vi "elevator_TP.vi"() -> ()   [LabVIEW 2020]
uses:
  State_enum.ctl
panel:
  out "Going down":bool
  out "Going up":bool
  out "Door closed":bool
  out "Alarm":bool
  out "Door open":bool
  out "Motor":bool
  out "state":T1
  in  "Stop Button":bool
  in  "1":bool
  in  "2":bool
  in  "3":bool
  out "Elevator":i8(slide) scale=0.0..2.0
  out "Destination floor":i32
  # "Current floor"
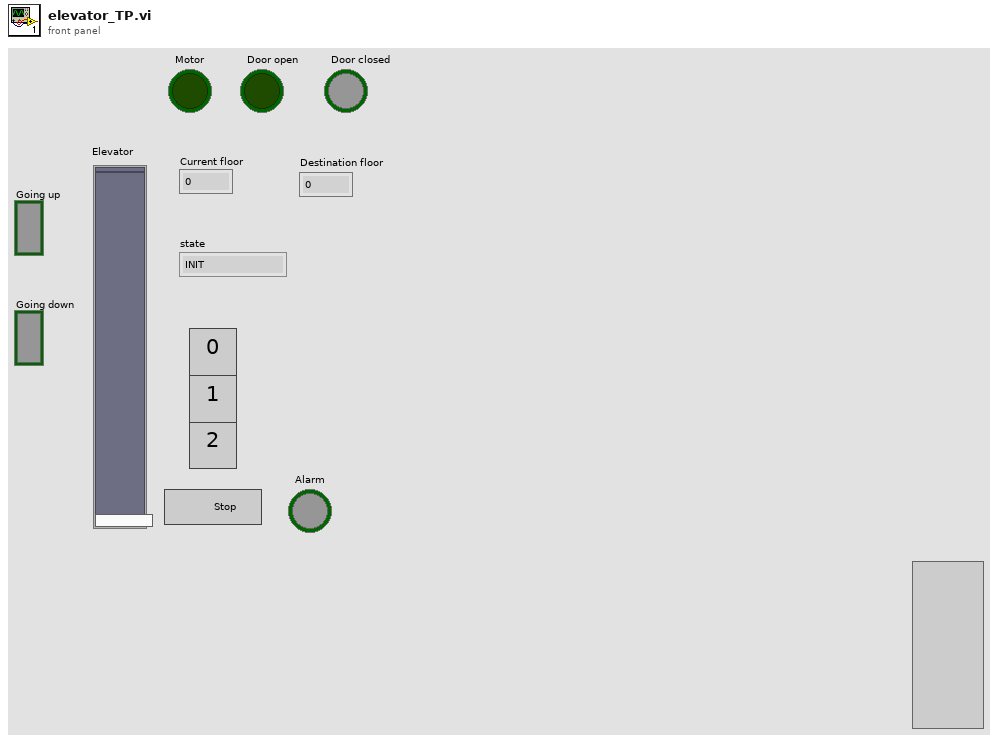
[diagram p1: front panel]
types:
  T1 = typedef "State_enum.ctl" = enum16{"INIT", "ATTENTE", "DEPLACEMENT", "PORTE_OUVERTE", "PORTE_FERMEE", "ARRET_URGENCE"}
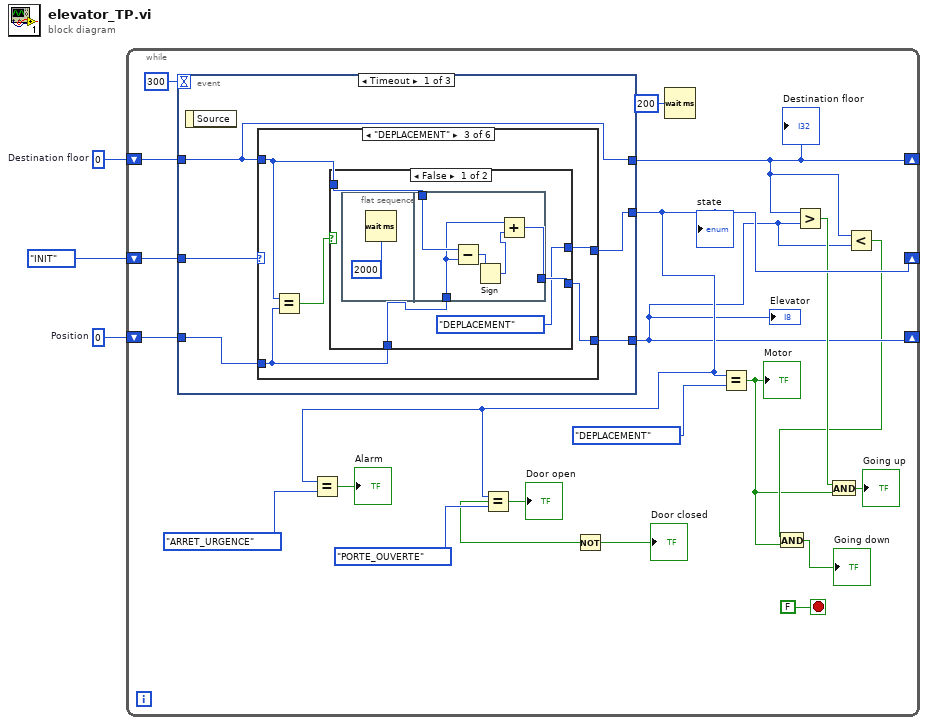
[diagram p0: block diagram]
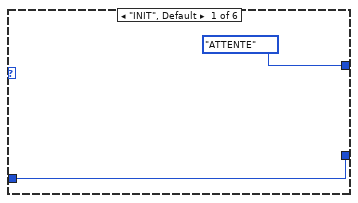
[diagram p2: hidden frame]
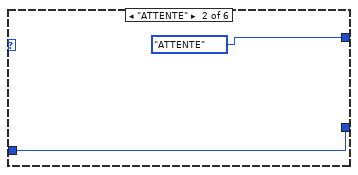
[diagram p3: hidden frame]
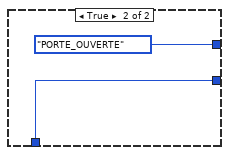
[diagram p4: hidden frame]
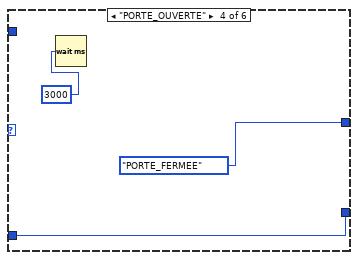
[diagram p5: hidden frame]
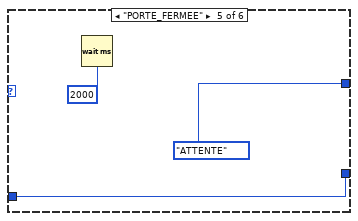
[diagram p6: hidden frame]
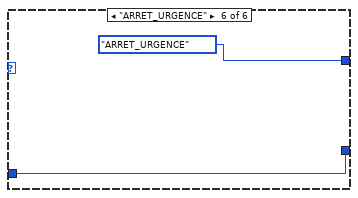
[diagram p7: hidden frame]
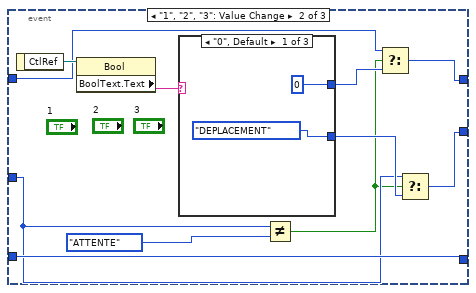
[diagram p8: hidden frame]
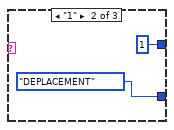
[diagram p9: hidden frame]
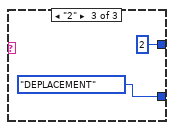
[diagram p10: hidden frame]
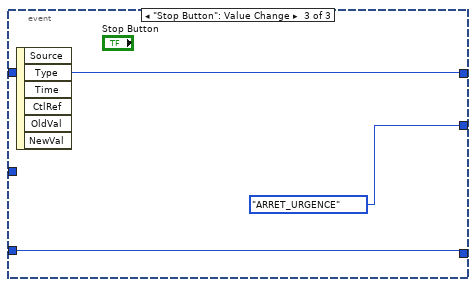
[diagram p11: hidden frame]
diagram:
  w2 = 0  # Position
  w3 = 0  # Destination floor
  n1 = while {
    shift-right: [w8] -> _
    shift-left: w3 -> [w20]
    shift-right: [w7] -> _
    shift-left: w2 -> [w21]
    shift-right: [w13] -> _
    shift-left: State_enum."INIT" ("state") -> [w22]
    stop <- FALSE stop-if-true
    n2 = event shown="[0] Timeout" {
      selector: _ -> [_ _ _]
      dyn-events: _ -> [_ _ _]
      timeout: 300 -> [_ _ _]
      tunnel: [w24 w62 w76] -> w8
      tunnel: w22 -> [w28 w60 _]
      tunnel: w21 -> [w27 w66 w75]
      tunnel: [w26 w66 w75] -> w7
      tunnel: [w25 w58 State_enum."ARRET_URGENCE" ("state")] -> w13
      tunnel: w20 -> [w24 w63 w76]
      event Timeout {
        n3 = event-data() -> ()  [unwired: 1 in, 1 out]
        n4 = case shown="\"DEPLACEMENT\"" w28 {
          tunnel: [w30 w32 w33 w52 w54 w56] -> w26
          tunnel: w24 -> [_ _ w35 _ _ _]
          tunnel: [State_enum."ATTENTE" ("state") State_enum."ATTENTE" ("state") w37 State_enum."PORTE_FERMEE" ("state") State_enum."ATTENTE" ("state") State_enum."ARRET_URGENCE" ("state")] -> w25
          tunnel: w27 -> [w30 w32 w34 w52 w54 w56]
          frame "INIT", Default {
          }
          frame "ATTENTE" {
          }
          frame "DEPLACEMENT" {
            n5 = Equal?(x=w35, y=w34) -> (x = y?=w36:bool)
            n6 = case shown="False" w36 {
              tunnel: [State_enum."DEPLACEMENT" ("state") State_enum."PORTE_OUVERTE" ("state")] -> w37
              tunnel: w34 -> [w40 w48]
              tunnel: w35 -> [w41 _]
              tunnel: [w39 w48] -> w33
              frame False {
                n7 = flat-sequence {
                  tunnel: w41 -> [w47]
                  tunnel: w40 -> [w44]
                  tunnel: [w43] -> _
                  tunnel: [w43] -> w39
                  frame #0 {
                    n8 = Wait (ms)(milliseconds to wait=u32 2000) -> ()  [unwired: 1 out]
                  }
                  frame #1 {
                    n9 = Subtract(x=w47, y=w44) -> (x-y=w46:i32)
                    n10 = Sign(1:w46) -> (0:w45:i32)
                    n11 = Add(x=w44, y=w45) -> (x+y=w43:i32)
                  }
                }
              }
              frame True {
              }
            }
          }
          frame "PORTE_OUVERTE" {
            n12 = Wait (ms)(milliseconds to wait=u32 3000) -> ()  [unwired: 1 out]
          }
          frame "PORTE_FERMEE" {
            n13 = Wait (ms)(milliseconds to wait=u32 2000) -> ()  [unwired: 1 out]
          }
          frame "ARRET_URGENCE" {
          }
        }
      }
      event "1", "2", "3": Value Change {
        n14 = event-data() -> ("CtlRef"=w68:refnum<vi>)  [unwired: 1 in]
        n15 = property class="Bool"(reference=w68) -> ("BoolText.Text"=w67:string)  [unwired: 1 in, 2 out]
        n16 = case shown="\"0\", Default" w67 {
          tunnel: [0 1 2] -> w64
          tunnel: [State_enum."DEPLACEMENT" ("state") State_enum."DEPLACEMENT" ("state") State_enum."DEPLACEMENT" ("state")] -> w61
          frame "0", Default {
          }
          frame "1" {
          }
          frame "2" {
          }
        }
        n17 = Not Equal?(x=w60, y=State_enum."ATTENTE" ("state")) -> (x != y?=w59:bool)
        n18 = Select(t=w63, s=w59, f=w64) -> (s? t:f=w62:i32)
        n19 = Select(t=w60, s=w59, f=w61) -> (s? t:f=w58:T1)
      }
      event "Stop Button": Value Change {
        n20 = event-data() -> ()  [unwired: 1 in, 6 out]
      }
    }
    "Elevator" <- w7
    "Destination floor" <- w8
    "state" <- w13
    n21 = Equal?(x=w13, y=State_enum."ARRET_URGENCE" ("state")) -> (x = y?=→"Alarm":bool)
    n22 = Equal?(x=w13, y=State_enum."PORTE_OUVERTE" ("state")) -> (x = y?=w12:bool)
    "Door open" <- w12
    n23 = Not(x=w12) -> (.not. x?=→"Door closed":bool)
    n24 = Wait (ms)(milliseconds to wait=u32 200) -> ()  [unwired: 1 out]
    n25 = Equal?(x=w13, y=State_enum."DEPLACEMENT" ("state")) -> (x = y?=w5:bool)
    "Motor" <- w5
    n26 = Greater?(x=w8, y=w7) -> (0:w10:bool)
    n27 = And(x=w10, y=w5) -> (x .and. y?=→"Going up":bool)
    n28 = Less?(x=w8, y=w7) -> (x < y?=w6:bool)
    n29 = And(x=w6, y=w5) -> (x .and. y?=→"Going down":bool)
  }
